vi "TxRollback_Core.vi"(8 "error in (no error)":errorcluster, 11 "DBC in":refnum<class "DBC.lvclass">) -> (0 "error out":errorcluster, 3 "DBC out":refnum<class "DBC.lvclass">)   [LabVIEW 2020, in "ORM_sqlite_jdp.lvlib" / "DBC.lvclass"]
uses:
  DBC.lvclass
  DBC.lvclass/DBC.ctl
  <vilib>/drjdpowell/SQLite Library/Transaction Helpers/Transaction.lvlib
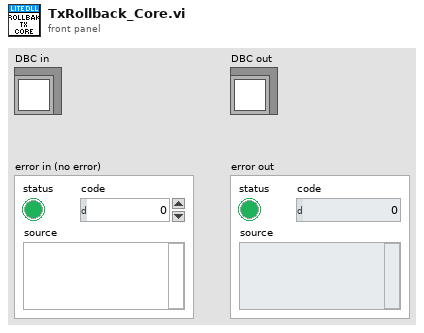
[diagram p1: front panel]
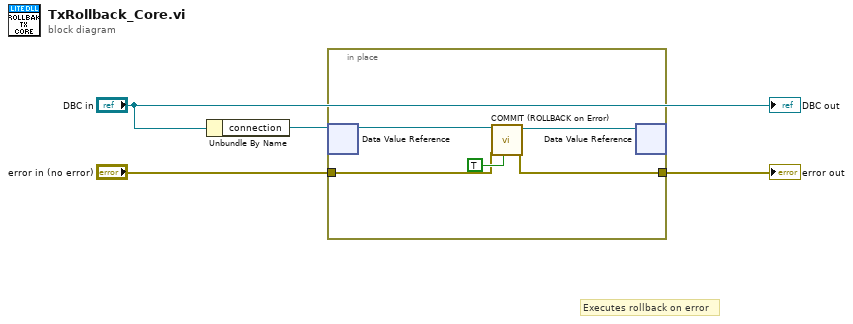
[diagram p0: block diagram]
diagram:
  # "Executes rollback on error"
  n1 = Unbundle By Name("DBC in") -> ("connection"=w3:refnum<data-value>)
  n2 = in-place {
    in-place-border: "error in (no error)" -> [w6]
    in-place-border: [w5] -> w1
    n3 = in-place-dvr #1(w3) -> (w9:refnum<class "Connection.lvclass">)  [unwired: 1 out]
    n4 = call <vilib>:"COMMIT (ROLLBACK on Error).vi"("ROLLBACK even if no error"=TRUE, "error in (no error)"=w6, "SQLite Connection in"=w9) -> ("error out"=w5:errorcluster, "SQLite Connection"=w8:refnum<class "Connection.lvclass">)  [unwired: 7 in]
    n5 = in-place-dvr #1(w8) -> ()  [unwired: 2 out]
  }
  "error out" <- w1
  "DBC out" <- "DBC in"
